vi "CFX.vi"(0 "CFX cmd":T6, 1 "CFX State":T7, 5 "CFX-config":T2={"neme"="上板机", "CFX Handle"="Cleaner", "Request IP"="amqp://192.168.1.10:5672", "User"="admin", "password"="123456", "Broker IP"="192.168.1.20", "Broker Port"="5672", "Publish Path"="/exchange/Cleaner", "SubPubish Path"="/queue/Broadcast-Cleaner", "Broadcast \nPublish Path"="/exchange/CFX.Host", "Broadcast Sub\npublish Path"="/queue/Broadcast-CFX.Host", "Target \nHandle lD"="CFX.Host", "target IP"="amqp://127.0.0.1", "unit verification"=TRUE, "heartbeat"=FALSE, "timeout period"=40.0}, 7 "CfxData":T1={"Vendor"="YXD", "UniqueIdentifier"="UID5620001", "FriendlyName"="SBJ", "ModelNumber"="SBJ_0001", "SerialNumber"="563210", "NumberofLanes"="2", "CodeIn"="", "CodeOut"="", "Unitldentifer"="", "PositionNumber"="", "PositionName"="", "OldState"="", "NewState"="", "OldStateDuration"="", "Faultcode"="", "Operatorldentifer"="", "LoginName"="", "RecipeName"="", "Revision"="", "Activate formula"="", "Description"=""}, 11 "Error In":errorcluster caption="错误输入", 12 "send?":bool) -> (6 "MessageCFX_out":string, 8 "CFX_Message_In":T3, 14 "ok?":bool, 15 "Error Out":errorcluster caption="错误输出")   [LabVIEW 2025]
uses:
  CFX_dll/CFX.dll
  ctl/CFX-cmd.ctl
  ctl/CfxTopic-cmd.ctl
  SubVI/table/1 model/a log/_myType runlog cmd.ctl
  ctl/CFX-config.ctl
  ctl/CFX_data.ctl
panel:
  out "QueueName":string
  out "IsOpenRequest":bool
  out "IsOpen":bool
  in  "CFX.Host?":bool
  in  "enable?":bool
  out "TraceMessage_EVE":refnum<k27>
  out "TraceMessage":string
  out "AooLog":refnum<k24>
  out "TestSubscribeChannel":bool
  out "TestPublishChannel":bool
  out "log":string
  out "error out":errorcluster
  out "objAMQP_MSG":refnum<k27>
  out "Connection":T4 {"ConnectionEstablished" items=["ConnectionEstablished", "ConnectionFailed", "ConnectionInterrupted", "ConnectionClosed"]}
  out "objAMQP_Request":refnum<k27>
  out "SubscribeChannel":refnum<k24>
  out "return":T5={"CFXHandle"="Cleaner", "RequestNetworkUri"="amqp://10.33.191.97:5672", "RequestTargetAddress"="/queue/Cleaner", "CFX_Message_In"={"Message_Name"="", "Message_Content"=""}, "CFX_Message_out"={"Message_Name"="", "Message_Content"=""}, "CFX_data"=refnum}
  out "FromListener":string
  in  "EndpointInformation":string
  in  "NewState":i32(ring)=1000 items=["PRD"=1000, "PRD_RegularWork"=1100, "PRD_WorkForThirdParties"=1200, "PRD_Rework"=1300, "PRD_Engineering"=1400, "SBY"=2000, "SBY_NoOperator"=2100, "SBY_NoProduct"=2200, "SBY_NoSupportTool"=2300, "SBY_AssociatedClusterModuleDown"=2400, "SBY_NoHost"=2500, "ENG"=3000, "ENG_ProcessExperiments"=3100, "ENG_EquipmentExperiments"=3200, "SDT"=4000, "SDT_UserMaintenanceDelay"=4100, "SDT_SuppliedMaintenanceDelay"=4200, "SDT_PreventiveMaintenance"=4300, "SDT_ChangeOfConsumables"=4400, "SDT_Setup"=4500, "SDT_ProductionTest"=4600, "SDT_FacilitiesRelated"=4700, "USD"=5000, "USD_UserMaintentanceDelay"=5100, "USD_SuppliedMaintenanceDelay"=5200, "USD_Repair"=5300, "USD_OutOfSpecInputMaterial"=5400, "USD_ChangeOfConsumables"=5500, "USD_FacilitiesRelated"=5600, "NST"=6000, "NST_UnworkedShifts"=6100, "NST_EquipmentInstallation"=6200, "NST_EquipmentModifications"=6300, "NST_OfflineTraining"=6400, "NST_ShutdownAndStartup"=6500]
  in  "Broker Url":string="amqp://admin:123456@10.33.191.54:5672"
  out "PublishChannel":refnum<k24>
  in  "rngNewState":i32(ring) items=["PRD"=1000, "PRD_RegularWork"=1100, "PRD_WorkForThirdParties"=1200, "PRD_Rework"=1300, "PRD_Engineering"=1400, "SBY"=2000, "SBY_NoOperator"=2100, "SBY_NoProduct"=2200, "SBY_NoSupportTool"=2300, "SBY_AssociatedClusterModuleDown"=2400, "SBY_NoHost"=2500, "ENG"=3000, "ENG_ProcessExperiments"=3100, "ENG_EquipmentExperiments"=3200, "SDT"=4000, "SDT_UserMaintenanceDelay"=4100, "SDT_SuppliedMaintenanceDelay"=4200, "SDT_PreventiveMaintenance"=4300, "SDT_ChangeOfConsumables"=4400, "SDT_Setup"=4500, "SDT_ProductionTest"=4600, "SDT_FacilitiesRelated"=4700, "USD"=5000, "USD_UserMaintentanceDelay"=5100, "USD_SuppliedMaintenanceDelay"=5200, "USD_Repair"=5300, "USD_OutOfSpecInputMaterial"=5400, "USD_ChangeOfConsumables"=5500, "USD_FacilitiesRelated"=5600, "NST"=6000, "NST_UnworkedShifts"=6100, "NST_EquipmentInstallation"=6200, "NST_EquipmentModifications"=6300, "NST_OfflineTraining"=6400, "NST_ShutdownAndStartup"=6500]
  # "此端点的唯一 CFX 句柄。"
  # "节点队列名"
  # "amqp://10.33.191.64:5672"
  # "amqp://localhost:5672"
  # "Laser"
  # "amqp://192.168.1.20:5672"
  # "AMQP 源或目标的网络地址。可以包括 user 和 port 信息 标准 Uri 格式。（例如：amqps://user1:password1@myamqpbroker.company1.com、amqp://broker3.company1.com、 amqps://myamqpbroker.company1.com:8856 等）。"
  # "本地消息源\nRequest Source"
  # "代理层\nBroker"
  # "请求目标\nRequest Target"
  # "可配置项"
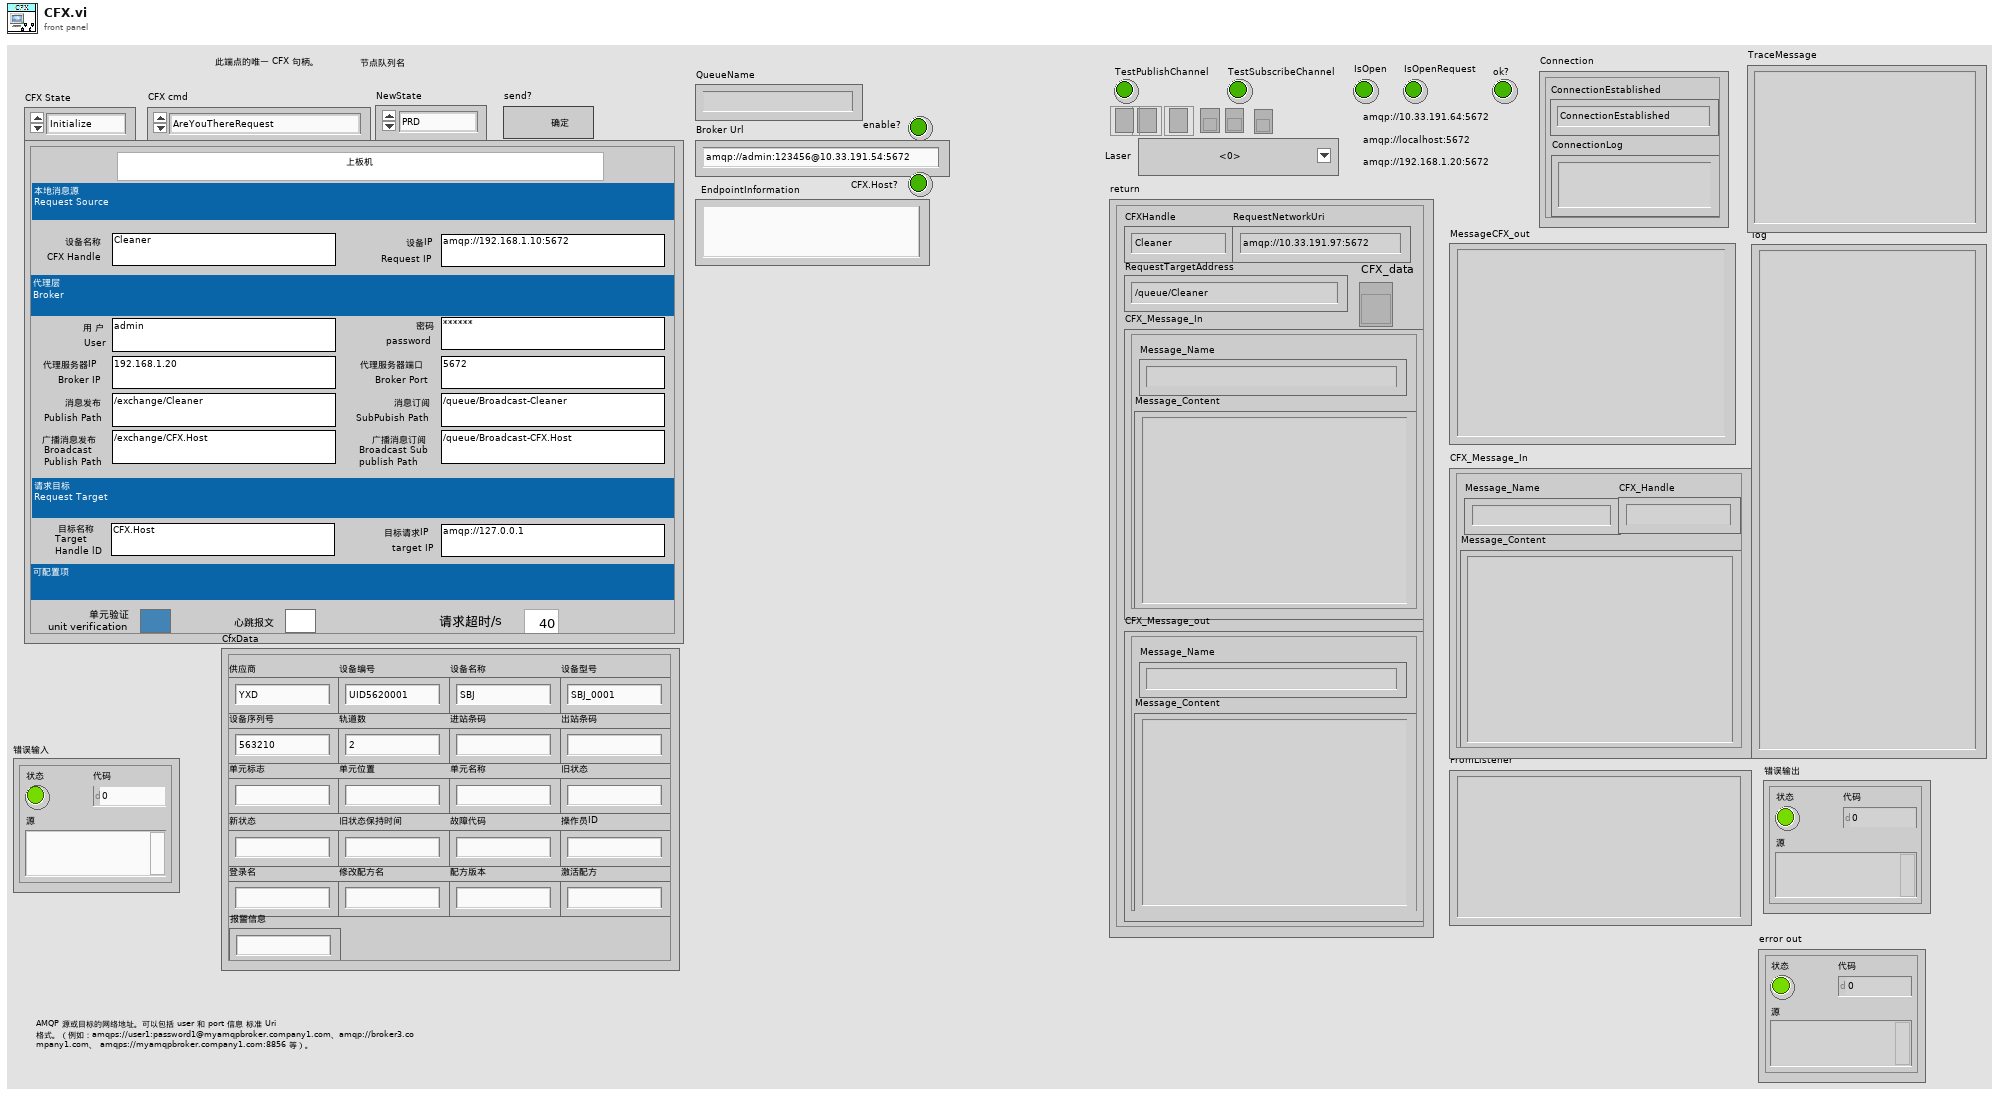
[diagram p1: front panel]
types:
  T1 = typedef "CFX_data.ctl" = cluster{"Vendor":string, "UniqueIdentifier":string, "FriendlyName":string, "ModelNumber":string, "SerialNumber":string, "NumberofLanes":string, "CodeIn":string, "CodeOut":string, "Unitldentifer":string, "PositionNumber":string, "PositionName":string, "OldState":string, "NewState":string, "OldStateDuration":string, "Faultcode":string, "Operatorldentifer":string, "LoginName":string, "RecipeName":string, "Revision":string, "Activate formula":string, "Description":string}
  T2 = typedef "CFX-config.ctl" = cluster{"neme":string, "CFX Handle":string, "Request IP":string, "User":string, "password":string, "Broker IP":string, "Broker Port":string, "Publish Path":string, "SubPubish Path":string, "Broadcast \nPublish Path":string, "Broadcast Sub\npublish Path":string, "Target \nHandle lD":string, "target IP":string, "unit verification":bool, "heartbeat":bool, "timeout period":dbl}
  T3 = cluster{"Message_Name":string, "CFX_Handle":string, "Message_Content":string}
  T4 = cluster{"ConnectionEstablished":i32, "ConnectionLog":string}
  T5 = cluster{"CFXHandle":string, "RequestNetworkUri":string, "RequestTargetAddress":string, "CFX_Message_In":cluster{"Message_Name":string, "Message_Content":string}, "CFX_Message_out":cluster{"Message_Name":string, "Message_Content":string}, "CFX_data":refnum<vi>}
  T6 = typedef "CfxTopic-cmd.ctl" = enum16{"AreYouThereRequest", "AreYouThereResponse", "EndpointConnected", "EndpointShuttingDown", "GetEndpointInformationRequest", "GetEndpointInformationResponse", "Heartbeat", "NotSupportedResponse", "WhoIsThereRequest", "WhoIsThereResponse", "UnitArrived", "UnitsDeparted", "StationStateChanged", "FaultOccurred", "FaultCleared", "OperatorActivated", "OperatorDeactivated", "RecipeModified", "RecipeActived", "ActivateRecipeRequest", "ActivateRecipeResponse"}
  T7 = typedef "CFX-cmd.ctl" = enum16{"Initialize", "Event", "Connection test", "OpenConnection", "Idle", "Shutdown", "WorkComplete", "StationStateChanged", "MaterialsApplied", "CFX", "Hermes"}
  T8 = typedef "_myType runlog cmd.ctl" = enum16{"init", "push (-1: error)", "push (0: user)", "push (1: logical)", "push (2: driver)", "push (3: lib-core)", "push (4: reserved)", "pop", "more?"}
  T9 = typedef "LVStringsAndValuesArrayTypeDef_I32.ctl" = cluster{"String":string, "Value":i32}[]
  T10 = cluster{"Message_Name":string, "Message_Content":string}
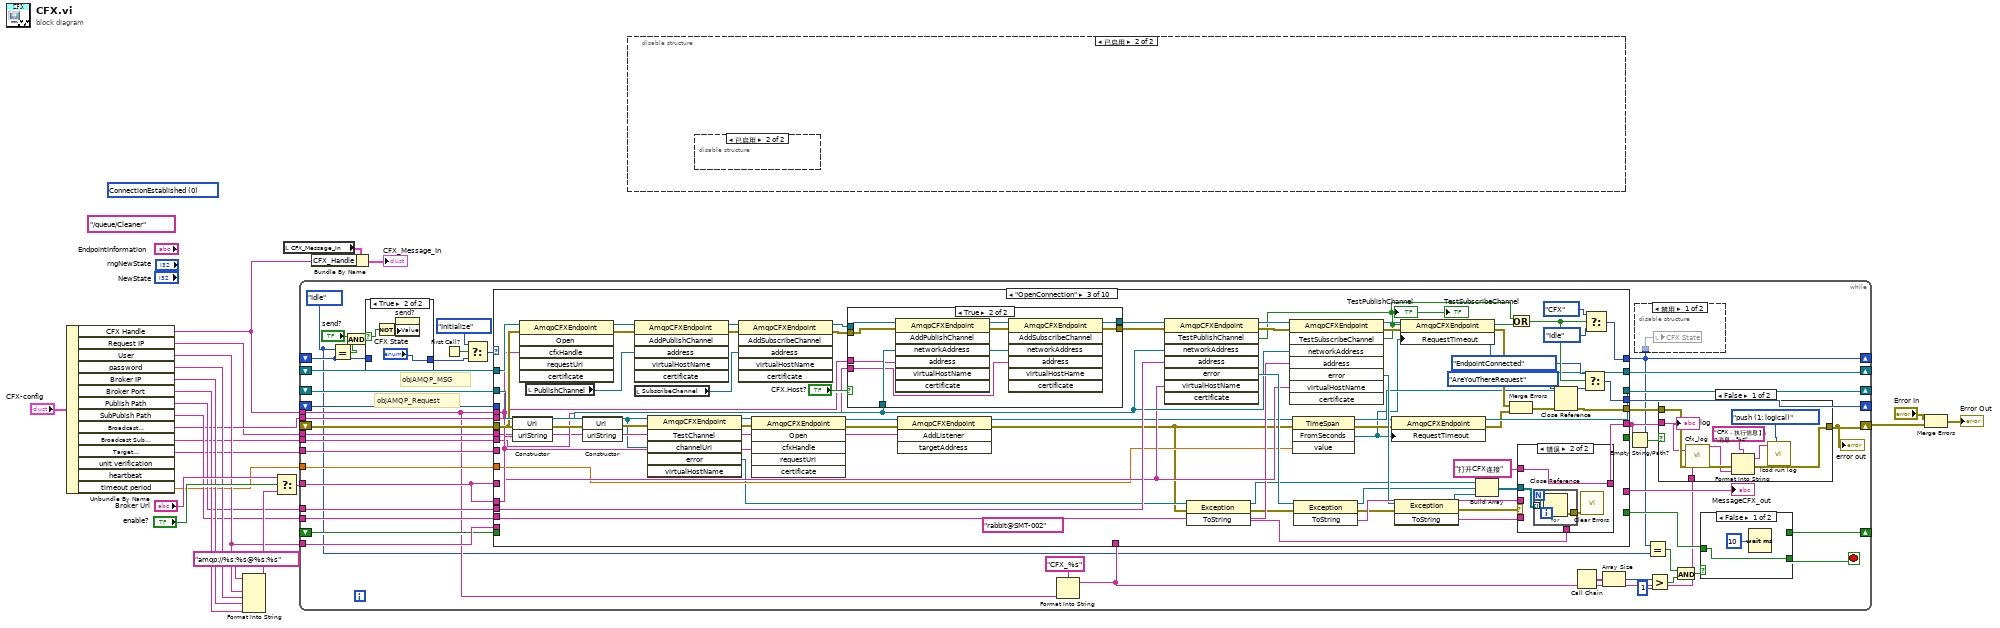
[diagram p0: block diagram]
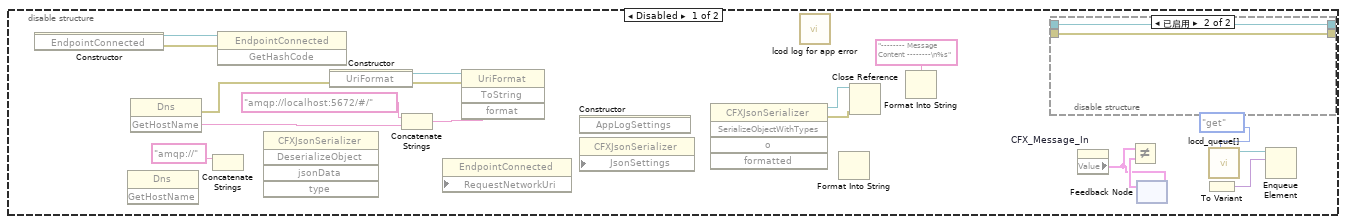
[diagram p2: hidden frame]
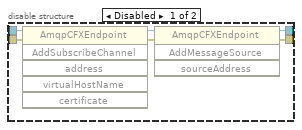
[diagram p3: hidden frame]
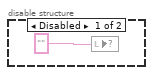
[diagram p4: hidden frame]
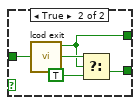
[diagram p7: hidden frame]
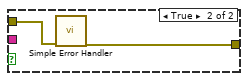
[diagram p8: hidden frame]
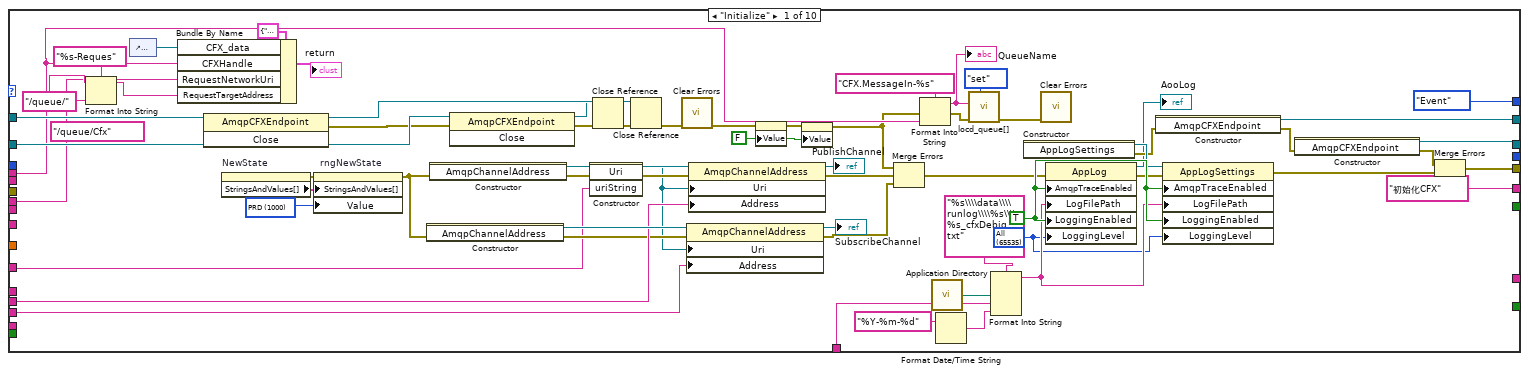
[diagram p9: hidden frame]
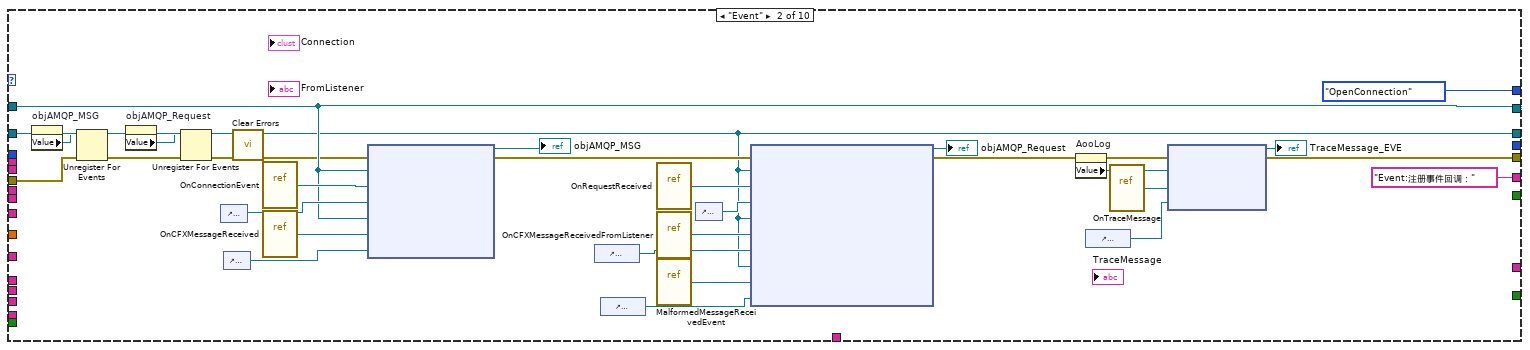
[diagram p10: hidden frame]
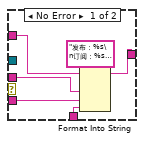
[diagram p12: hidden frame]
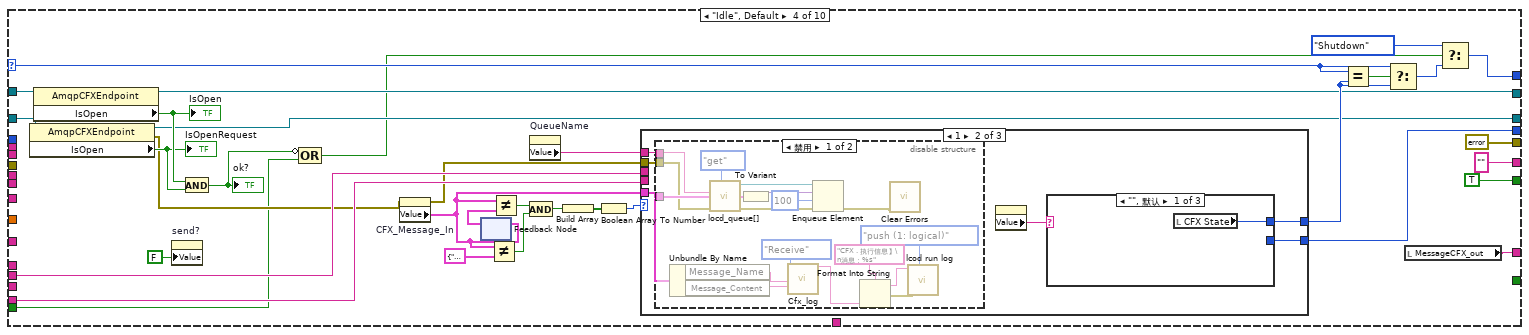
[diagram p13: hidden frame]
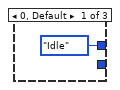
[diagram p14: hidden frame]
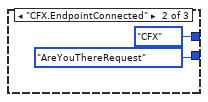
[diagram p16: hidden frame]
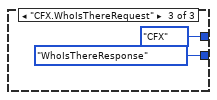
[diagram p17: hidden frame]
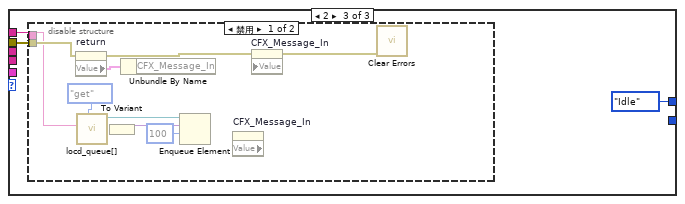
[diagram p18: hidden frame]
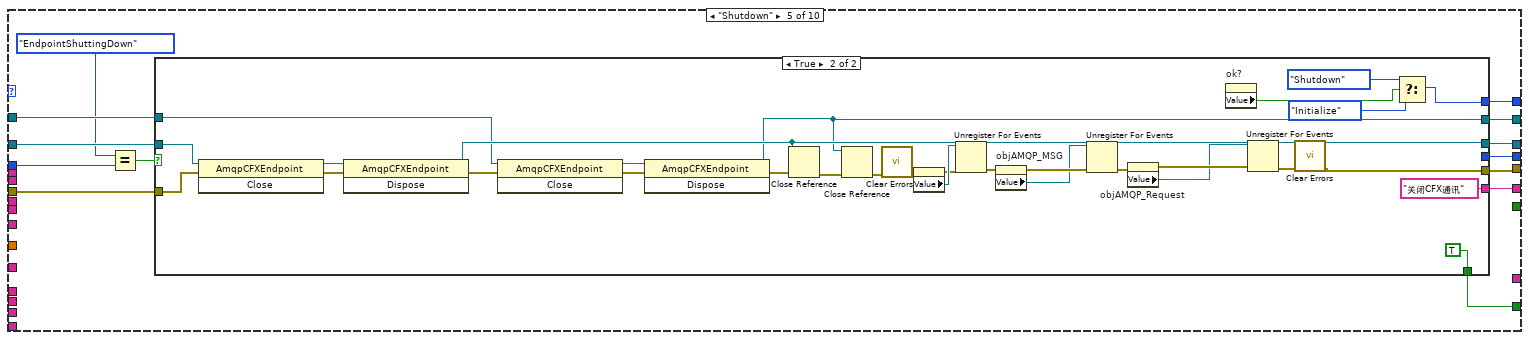
[diagram p20: hidden frame]
diagram:
  (unwired) "/queue/Cleaner" ("RequestTargetAddress")
  (unwired) 0 items=["ConnectionEstablished", "ConnectionFailed", "ConnectionInterrupted", "ConnectionClosed"] ("ConnectionEstablished")
  n1 = Unbundle By Name("CFX-config") -> ("CFX Handle"=w3:string, "Request IP"=w6:string, "User"=w16:string, "password"=w15:string, "Broker IP"=w14:string, "Broker Port"=w13:string, "Publish Path"=w12:string, "SubPubish Path"=w11:string, "Broadcast \nPublish Path"=w10:string, "Broadcast Sub\npublish Path"=w9:string, "Target \nHandle lD"=w8:string, "timeout period"=w7:dbl)  [unwired: 2 out]
  n2 = Format Into String(format string="amqp://%s:%s@%s:%s" ("格式字符串"), w16, w15, w14, w13) -> (resulting string=w18:string)  [unwired: 2 in, 1 out]
  n3 = Select(t="Broker Url", s="enable?", f=w18) -> (s? t:f=w5:string)
  n4 = local read "CFX_Message_In"() -> (w2:T3)
  n5 = while {
    shift-right: [w41] -> _
    shift-left: _ -> [w27]
    shift-right: [w66] -> _
    shift-left: _ -> [w67]
    shift-right: [w63] -> _
    shift-left: _ -> [w62]
    shift-right: [w58] -> w4
    shift-left: _ -> [w52]
    shift-right: [w57] -> _
    shift-left: _ -> [w59]
    tunnel: w5 -> [w53]
    tunnel: w11 -> [w56]
    tunnel: w12 -> [w55]
    tunnel: w3 -> [w32]
    tunnel: w16 -> [w54]
    tunnel: w6 -> [w51]
    tunnel: w10 -> [w50]
    tunnel: w9 -> [w49]
    tunnel: w8 -> [w48]
    tunnel: w7 -> [w47]
    shift-right: [w28] -> _
    shift-left: _ -> [w34]
    stop <- w42 stop-if-true
    w26 = CFX-cmd."Idle" ("CFX State")
    # "objAMQP_Request"
    # "objAMQP_MSG"
    n6 = Equal?(x=w26, y=w27) -> (x = y?=w24:bool)
    n7 = And(x="send?", y=w24) -> (x .and. y?=w25:bool)
    n8 = case shown="True" w25 {
      selector: w25 -> [_ w71]
      tunnel: w27 -> [w69 _]
      tunnel: [w69 "CFX State"] -> w31
      frame False {
      }
      frame True {
        n9 = Not(x=w71) -> (.not. x?=w70:bool)
        n10 = property on="send?" class="Bool (严格)"("Value"=w70) -> ()  [unwired: 2 in, 2 out]
      }
    }
    n11 = First Call?() -> (First Call?: T/F=w36:bool)
    n12 = Select(t=CFX-cmd."Initialize" ("CFX State"), s=w36, f=w31) -> (s? t:f=w35:T7)
    n13 = Format Into String(format string="CFX_%s" ("log_path"), w32) -> (resulting string=w30:string)  [unwired: 2 in, 1 out]
    n14 = case shown="\"OpenConnection\"" w35 {
      selector: w35 -> [_ _ _ w306 _ _ _ _ _ _]
      tunnel: [_ _ _ _ w352 _ _ _ _ _] -> w43
      tunnel: w67 -> [w131 w161 w250 w294 w360 w412 w441 w467 w508 w527]
      tunnel: [w138 w161 w203 w293 w355 w411 w439 w466 w506 w526] -> w66
      tunnel: [w132 w173 w217 errorcluster {"status"=FALSE, "code"=0, "source"=""} ("error out") w353 w408 w436 w465 w518 w525] -> w65
      tunnel: [_ _ _ w305 _ w403 w428 w452 w501 w524] -> w64
      tunnel: [_ _ _ TRUE _ _ _ _ _ _] -> _
      tunnel: ["初始化CFX" ("格式字符串") "Event:注册事件回调：" ("SerializeObjectWithTypes") w242 "" ("SerializeObjectWithTypes") w359 w400 w428 w451 w512 w524] -> w61
      tunnel: [CFX-cmd."Event" ("CFX State") CFX-cmd."OpenConnection" ("CFX State") w210 w284 w358 CFX-cmd."Idle" ("CFX State") CFX-cmd."Idle" ("CFX State") CFX-cmd."Idle" ("CFX State") w487 CFX-cmd."Idle" ("CFX State")] -> w41
      tunnel: [w137 w160 w234 w288 w354 w397 w425 w448 w507 w521] -> w63
      tunnel: w62 -> [w130 w160 w246 w295 w356 w397 w425 w448 w507 w521]
      tunnel: w52 -> [_ w168 w221 _ w357 w398 w426 w449 w509 w522]
      tunnel: w59 -> [_ _ _ _ w351 _ _ _ w491 _]
      tunnel: [_ _ w206 w300 w348 _ _ _ w486 _] -> w57
      tunnel: w53 -> [w93 _ _ _ _ _ _ _ _ _]
      tunnel: w56 -> [w117 _ w199 _ _ _ _ _ _ _]
      tunnel: w55 -> [w116 _ w230 w297 _ _ _ _ _ _]
      tunnel: w32 -> [w96 _ w213 _ _ _ _ _ w484 _]
      tunnel: w54 -> [_ _ _ w296 _ _ _ _ _ _]
      tunnel: w53 -> [_ _ w229 _ _ _ _ _ _ _]
      tunnel: w51 -> [w97 _ w196 _ _ _ _ _ _ _]
      tunnel: w50 -> [_ _ w201 _ _ _ _ _ _ _]
      tunnel: w49 -> [_ _ w200 _ _ _ _ _ _ _]
      tunnel: w48 -> [_ _ _ _ _ _ _ _ w483 _]
      tunnel: w47 -> [_ _ w198 _ _ _ _ _ _ _]
      tunnel: w34 -> [_ _ _ w287 _ _ _ _ _ _]
      tunnel: w30 -> [w95 _ _ _ _ _ _ _ _ _]
      frame "Initialize" {
        (unwired) "/queue/Cfx" ("RequestTargetAddress")
        w121 = FALSE ("TestPublishChannel")
        w134 = 65535 items=["Debug"=1, "Info"=2, "Warn"=4, "Error"=8, "All"=65535] ("LoggingLevel")
        w136 = TRUE ("LoggingEnabled")
        w149 = 1000 items=["PRD"=1000, "PRD_RegularWork"=1100, "PRD_WorkForThirdParties"=1200, "PRD_Rework"=1300, "PRD_Engineering"=1400, "SBY"=2000, "SBY_NoOperator"=2100, "SBY_NoProduct"=2200, "SBY_NoSupportTool"=2300, "SBY_AssociatedClusterModuleDown"=2400, "SBY_NoHost"=2500, "ENG"=3000, "ENG_ProcessExperiments"=3100, "ENG_EquipmentExperiments"=3200, "SDT"=4000, "SDT_UserMaintenanceDelay"=4100, "SDT_SuppliedMaintenanceDelay"=4200, "SDT_PreventiveMaintenance"=4300, "SDT_ChangeOfConsumables"=4400, "SDT_Setup"=4500, "SDT_ProductionTest"=4600, "SDT_FacilitiesRelated"=4700, "USD"=5000, "USD_UserMaintentanceDelay"=5100, "USD_SuppliedMaintenanceDelay"=5200, "USD_Repair"=5300, "USD_OutOfSpecInputMaterial"=5400, "USD_ChangeOfConsumables"=5500, "USD_FacilitiesRelated"=5600, "NST"=6000, "NST_UnworkedShifts"=6100, "NST_EquipmentInstallation"=6200, "NST_EquipmentModifications"=6300, "NST_OfflineTraining"=6400, "NST_ShutdownAndStartup"=6500] ("NewState")
        n15 = Format Into String(format string="%s-Reques" ("格式字符串"), initial string="/queue/" ("RequestTargetAddress"), w96) -> (resulting string=w90:string)  [unwired: 1 in, 1 out]
        n16 = control-ref of="CfxData"() -> (w101:refnum<vi>)
        n17 = Bundle By Name(cluster=T5 {"CFXHandle"="Cleaner", "RequestNetworkUri"="amqp://192.168.1.10:5672", "RequestTargetAddress"="/queue/Cleaner", "CFX_Message_In"={"Message_Name"="", "Message_Content"=""}, "CFX_Message_out"={"Message_Name"="", "Message_Content"=""}, "CFX_data"=refnum} ("return"), "CFX_data"=w101, "CFXHandle"=w96, "RequestNetworkUri"=w97, "RequestTargetAddress"=w90) -> (→"return":T5)
        n18 = invoke class="AmqpCFXEndpoint" method="Close"(reference=w131) -> (reference out=w125:refnum<k24>, error out=w129:errorcluster)  [unwired: 2 in, 1 out]
        n19 = property on="NewState" class="Ring (严格)"() -> (error out=w148:errorcluster, "StringsAndValues[]"=w152:T9)  [unwired: 2 in, 1 out]
        n20 = property on="rngNewState" class="Ring (严格)"(error in=w148, "StringsAndValues[]"=w152, "Value"=w149) -> (error out=w123:errorcluster)  [unwired: 1 in, 1 out]
        n21 = constructor class="AmqpChannelAddress"(error in=w123) -> (reference out=w142:refnum<k24>, error out=w115:errorcluster)  [unwired: 2 in, 1 out]
        n22 = constructor class="AmqpChannelAddress"(error in=w123) -> (reference out=w147:refnum<k24>, error out=w151:errorcluster)  [unwired: 2 in, 1 out]
        n23 = invoke class="AmqpCFXEndpoint" method="Close"(reference=w130, error in=w129) -> (reference out=w124:refnum<k24>, error out=w128:errorcluster)  [unwired: 1 in, 1 out]
        n24 = constructor class="Uri"(error in=w151, "uriString"=w93) -> (reference out=w114:refnum<k24>, error out=w150:errorcluster)  [unwired: 2 in, 2 out]
        n25 = Close Reference(reference=w124, error in (no error)=w128) -> (error out=w127:errorcluster)
        n26 = Close Reference(reference=w125, error in (no error)=w127) -> (error out=w126:errorcluster)
        n27 = call <vilib>:"Clear Errors.vi"("error in (no error)"=w126) -> ("error out"=w113:errorcluster)  [unwired: 5 in, 1 out]
        n28 = property class="AmqpChannelAddress"(reference=w142, error in=w115, "Uri"=w114, "Address"=w117) -> (reference out=→"SubscribeChannel":refnum<k24>, error out=w140:errorcluster)
        n29 = property class="AmqpChannelAddress"(reference=w147, error in=w150, "Uri"=w114, "Address"=w116) -> (reference out=→"PublishChannel":refnum<k24>, error out=w141:errorcluster)
        n30 = property on="TestPublishChannel" class="Bool (严格)"(error in=w113, "Value"=w121) -> (error out=w122:errorcluster)  [unwired: 1 in, 1 out]
        n31 = property on="TestSubscribeChannel" class="Bool (严格)"(error in=w122, "Value"=w121) -> (error out=w92:errorcluster)  [unwired: 1 in, 1 out]
        n32 = Merge Errors(w92, w141, w140) -> (w104:errorcluster)
        n33 = Format Into String(format string="CFX.MessageIn-%s" ("格式字符串"), error in=w92, w96) -> (resulting string=w105:string, error out=w102:errorcluster)  [unwired: 1 in]
        "QueueName" <- w105
        n34 = call <vilib>:"Application Directory.vi"() -> ("Application Directory"=w146:path)
        n35 = Format Date/Time String(time format string (%c)="%Y-%m-%d" ("格式字符串")) -> (date/time string=w94:string)  [unwired: 2 in]
        n36 = call "locd_queue[].vi"("cmd"=enum16{"init", "get", "set", "end"}."set", "error in"=w102, "queue_name"=w105) -> ("error out"=w103:errorcluster)  [unwired: 4 in, 4 out]
        n37 = Format Into String(format string="%s\\\\data\\\\runlog\\\\%s\\\\%s_cfxDebig.txt" ("格式字符串"), w146, w95, w94) -> (resulting string=w135:string)  [unwired: 2 in, 1 out]
        n38 = constructor class="AppLogSettings"() -> (reference out=w133:refnum<k24>, error out=w120:errorcluster)  [unwired: 3 in, 1 out]
        n39 = call <vilib>:"Clear Errors.vi"("error in (no error)"=w103) -> ()  [unwired: 5 in, 2 out]
        n40 = property class="AppLog"(error in=w104, "AmqpTraceEnabled"=w136, "LogFilePath"=w135, "LoggingEnabled"=w136, "LoggingLevel"=w134) -> (reference out=→"AooLog":refnum<k24>, error out=w118:errorcluster)  [unwired: 1 in]
        n41 = constructor class="AmqpCFXEndpoint"(error in=w120) -> (reference out=w138:refnum<k24>, error out=w109:errorcluster)  [unwired: 2 in, 1 out]
        n42 = property class="AppLogSettings"(reference=w133, error in=w118, "AmqpTraceEnabled"=w136, "LogFilePath"=w135, "LoggingEnabled"=w136, "LoggingLevel"=w134) -> (error out=w110:errorcluster)  [unwired: 1 out]
        n43 = constructor class="AmqpCFXEndpoint"(error in=w109) -> (reference out=w137:refnum<k24>, error out=w108:errorcluster)  [unwired: 2 in, 1 out]
        n44 = Merge Errors(w108, w110) -> (w132:errorcluster)
      }
      frame "Event" {
        n45 = property on="objAMQP_MSG" class="Ref (严格)"() -> ("Value"=w155:refnum<k27>)  [unwired: 2 in, 2 out]
        n46 = Unregister For Events(event registration refnum=w155, error in=w168) -> (error out=w156:errorcluster)
        n47 = property on="objAMQP_Request" class="Ref (严格)"() -> ("Value"=w153:refnum<k27>)  [unwired: 2 in, 2 out]
        n48 = Unregister For Events(event registration refnum=w153, error in=w156) -> (error out=w154:errorcluster)
        n49 = control-ref of="Connection"() -> (w180:refnum<vi>)
        n50 = control-ref of="CFX_Message_In"() -> (w165:refnum<vi>)
        n51 = call <vilib>:"Clear Errors.vi"("error in (no error)"=w154) -> ("error out"=w157:errorcluster)  [unwired: 5 in, 1 out]
        n52 = vi-ref "OnConnectionEvent.vi"() -> ("vi reference"=w181:refnum<vi>)
        n53 = vi-ref "OnCFXMessageReceived.vi"() -> ("vi reference"=w166:refnum<vi>)
        n54 = node(w157, w161, w181, w180, w161, w166, w165) -> (→"objAMQP_MSG":refnum<k27>, w164:errorcluster)  [unwired: 1 in]
        n55 = control-ref of="FromListener"() -> (w162:refnum<vi>)
        n56 = control-ref of="FromListener"() -> (w158:refnum<vi>)
        n57 = vi-ref "OnRequestReceived.vi"() -> ("vi reference"=w179:refnum<vi>)
        n58 = vi-ref "OnCFXMessageReceivedFromListener.vi"() -> ("vi reference"=w163:refnum<vi>)
        n59 = vi-ref "MalformedMessageReceivedEvent.vi"() -> ("vi reference"=w159:refnum<vi>)
        n60 = control-ref of="return"() -> (w170:refnum<vi>)
        n61 = node(w164, w160, w179, w170, w160, w163, w162, w160, w159, w158) -> (→"objAMQP_Request":refnum<k27>, w167:errorcluster)  [unwired: 1 in]
        n62 = property on="AooLog" class="Ref (严格)"(error in=w167) -> (error out=w169:errorcluster, "Value"=w175:refnum<k24>)  [unwired: 1 in, 1 out]
        n63 = control-ref of="TraceMessage"() -> (w171:refnum<vi>)
        n64 = vi-ref "OnTraceMessage.vi"() -> ("vi reference"=w174:refnum<vi>)
        n65 = node(w169, w175, w174, w171) -> (→"TraceMessage_EVE":refnum<k27>, w173:errorcluster)  [unwired: 1 in]
      }
      frame "OpenConnection" {
        (unwired) "rabbit@SMT-002" ("sourceAddress")
        n66 = constructor class="Uri"(error in=w221, "uriString"=w229) -> (reference out=w228:refnum<k24>, error out=w226:errorcluster)  [unwired: 2 in, 2 out]
        n67 = invoke class="AmqpCFXEndpoint" method="Open"(reference=w250, error in=w221, "cfxHandle"=w213) -> (reference out=w225:refnum<k24>, error out=w224:errorcluster)  [unwired: 3 in, 4 out]
        n68 = local read "PublishChannel"() -> (w244:refnum<k24>)
        n69 = constructor class="Uri"(error in=w226, "uriString"=w196) -> (reference out=w183:refnum<k24>, error out=w194:errorcluster)  [unwired: 2 in, 2 out]
        n70 = local read "SubscribeChannel"() -> (w245:refnum<k24>)
        n71 = invoke class="AmqpCFXEndpoint" method="AddPublishChannel"(reference=w225, error in=w224, "address"=w244) -> (reference out=w249:refnum<k24>, error out=w248:errorcluster)  [unwired: 3 in, 4 out]
        n72 = invoke on="调用节点" class="AmqpCFXEndpoint" method="TestChannel"(reference=w246, error in=w194, "channelUri"=w183) -> (reference out=w185:refnum<k24>, error out=w184:errorcluster, "error"=w193:refnum<k24>)  [unwired: 3 in, 3 out]
        n73 = invoke class="AmqpCFXEndpoint" method="AddSubscribeChannel"(reference=w249, error in=w248, "address"=w245) -> (reference out=w222:refnum<k24>, error out=w214:errorcluster)  [unwired: 3 in, 4 out]
        n74 = invoke class="AmqpCFXEndpoint" method="Open"(reference=w185, error in=w184, "cfxHandle"=w213, "requestUri"=w183) -> (reference out=w231:refnum<k24>, error out=w195:errorcluster)  [unwired: 2 in, 4 out]
        n75 = case shown="True" "CFX.Host?" {
          tunnel: w228 -> [_ w261]
          tunnel: [w251 w260] -> w227
          tunnel: [w252 w259] -> w223
          tunnel: w222 -> [w252 w258]
          tunnel: w214 -> [w251 w255]
          tunnel: w201 -> [_ w254]
          tunnel: w200 -> [_ w253]
          frame False {
          }
          frame True {
            n76 = invoke class="AmqpCFXEndpoint" method="AddPublishChannel"(reference=w258, error in=w255, "networkAddress"=w261, "address"=w254) -> (reference out=w256:refnum<k24>, error out=w257:errorcluster)  [unwired: 3 in, 5 out]
            n77 = invoke class="AmqpCFXEndpoint" method="AddSubscribeChannel"(reference=w256, error in=w257, "networkAddress"=w261, "address"=w253) -> (reference out=w259:refnum<k24>, error out=w260:errorcluster)  [unwired: 3 in, 5 out]
          }
        }
        n78 = invoke on="调用节点" class="AmqpCFXEndpoint" method="AddListener"(reference=w231, error in=w195, "targetAddress"=w196) -> (reference out=w197:refnum<k24>, error out=w192:errorcluster)  [unwired: 1 in, 2 out]
        n79 = invoke on="调用节点" class="AmqpCFXEndpoint" method="TestPublishChannel"(reference=w223, error in=w227, "networkAddress"=w228, "address"=w230, "virtualHostName"=w213) -> (reference out=w243:refnum<k24>, error out=w233:errorcluster, "TestPublishChannel"=w212:bool, "error"=w240:refnum<k24>)  [unwired: 3 in, 4 out]
        "TestPublishChannel" <- w212
        n80 = invoke class="Exception" method="ToString"(reference=w193, error in=w192) -> (reference out=w189:refnum<k24>, error out=w191:errorcluster, "ToString"=w190:string)  [unwired: 1 in]
        n81 = invoke on="调用节点" class="AmqpCFXEndpoint" method="TestSubscribeChannel"(reference=w243, error in=w233, "networkAddress"=w228, "address"=w199, "virtualHostName"=w213) -> (reference out=w241:refnum<k24>, error out=w219:errorcluster, "TestSubscribeChannel"=w211:bool, "error"=w237:refnum<k24>)  [unwired: 3 in, 4 out]
        "TestSubscribeChannel" <- w211
        n82 = invoke class="TimeSpan" method="FromSeconds"(error in=w192, "value"=w198) -> (reference out=w216:refnum<k24>, error out=w218:errorcluster, "FromSeconds"=w202:refnum<k24>)  [unwired: 2 in, 1 out]
        n83 = invoke class="Exception" method="ToString"(reference=w240, error in=w191) -> (reference out=w188:refnum<k24>, error out=w238:errorcluster, "ToString"=w239:string)  [unwired: 1 in]
        n84 = property on="属性节点" class="AmqpCFXEndpoint"(reference=w197, error in=w218, "RequestTimeout"=w202) -> (reference out=w234:refnum<k24>, error out=w220:errorcluster)
        n85 = invoke class="Exception" method="ToString"(reference=w237, error in=w238) -> (reference out=w187:refnum<k24>, error out=w235:errorcluster, "ToString"=w236:string)  [unwired: 1 in]
        n86 = property on="属性节点" class="AmqpCFXEndpoint"(reference=w241, "RequestTimeout"=w202) -> (reference out=w203:refnum<k24>)  [unwired: 1 in, 1 out]
        n87 = Build Array(w189, w188, w187) -> (w186:refnum<k24>[])
        n88 = Merge Errors(w219, w220) -> (w232:errorcluster)
        n89 = Or(x=w212, y=w211) -> (x .or. y?=w207:bool)
        n90 = case shown="错误" w235 {
          tunnel: "打开CFX连接" ("格式字符串") -> [w267 w270]
          tunnel: [w266 w270] -> w242
          tunnel: w239 -> [w264 _]
          tunnel: w236 -> [w263 _]
          tunnel: w190 -> [w262 _]
          tunnel: w186 -> [_ w269]
          frame No Error {
            n91 = Format Into String(format string="发布：%s\n订阅：%s\n监听监控：%s" ("格式字符串"), initial string=w267, w264, w263, w262) -> (resulting string=w266:string)  [unwired: 1 in, 1 out]
          }
          frame Error {
            n92 = for {
              tunnel: w269 -> [w272] mode=indexing
              tunnel: [w271] -> w268
              n93 = Close Reference(reference=w272) -> (error out=w271:errorcluster)  [unwired: 1 in]
            }
            n94 = call <vilib>:"Clear Errors.vi"("error in (no error)"=w268) -> ()  [unwired: 5 in, 2 out]
          }
        }
        n95 = Close Reference(reference=w216, error in (no error)=w232) -> (error out=w217:errorcluster)
        n96 = Select(t=CfxTopic-cmd."EndpointConnected" ("CFX cmd"), s=w207, f=CfxTopic-cmd."AreYouThereRequest") -> (s? t:f=w206:T6)
        n97 = Select(t=CFX-cmd."CFX" ("CFX State"), s=w207, f=CFX-cmd."Idle" ("CFX State")) -> (s? t:f=w210:T7)
      }
      frame "Idle", Default {
        n98 = property on="属性节点" class="AmqpCFXEndpoint"(reference=w295) -> (reference out=w288:refnum<k24>, error out=w290:errorcluster, "IsOpen"=w291:bool)  [unwired: 1 in]
        "IsOpenRequest" <- w291
        n99 = property on="属性节点" class="AmqpCFXEndpoint"(reference=w294) -> (reference out=w293:refnum<k24>, "IsOpen"=w292:bool)  [unwired: 1 in, 1 out]
        "IsOpen" <- w292
        n100 = property on="send?" class="Bool (严格)"("Value"=FALSE ("send?")) -> ()  [unwired: 2 in, 2 out]
        n101 = And(x=w292, y=w291) -> (x .and. y?=w273:bool)
        "ok?" <- w273
        n102 = Compound Arithmetic op=OR ("复合运算")(invert w273, w287) -> (w274:bool)
        n103 = property on="CFX_Message_In" class="Clust (严格)"(error in=w290) -> (error out=w289:errorcluster, "Value"=w279:T3)  [unwired: 1 in, 1 out]
        n104 = feedback-in #1(w279) -> ()
        n105 = feedback #1() -> (w298:T3)  [unwired: 1 in]
        n106 = Not Equal?(x=w279, y=T3 {"Message_Name"="", "CFX_Handle"="", "Message_Content"=""} ("CFX_Message_In")) -> (x != y?=w277:bool)
        n107 = Not Equal?(x=w279, y=w298) -> (x != y?=w283:bool)
        n108 = And(x=w283, y=w277) -> (x .and. y?=w278:bool)
        n109 = property on="QueueName" class="Str"() -> ("Value"=w280:string)  [unwired: 2 in, 2 out]
        n110 = Build Array(w278) -> (w281:bool[])
        n111 = Boolean Array To Number(Boolean array=w281) -> (number=w282:u32)
        n112 = case shown="1" w282 {
          tunnel: [_ w313 _] -> w300
          tunnel: [CFX-cmd."Idle" ("CFX State") w312 CFX-cmd."Idle" ("CFX State")] -> w299
          tunnel: w297 -> [_ _ _]
          tunnel: w296 -> [_ _ _]
          tunnel: w279 -> [_ w310 _]
          tunnel: w289 -> [_ w308 w338]
          tunnel: w280 -> [_ w309 w336]
          frame 0, Default {
          }
          frame 1 {
            n113 = disable-structure shown="禁用" {
              disable-tunnel: w310 -> [w326 _]
              disable-tunnel: w309 -> [w316 _]
              disable-tunnel: w308 -> [w315 _]
              frame Disabled {
                n114 = Unbundle By Name(w326) -> ("Message_Name"=w325:string, "Message_Content"=w324:string)
                n115 = call "locd_queue[].vi"("cmd"=enum16{"init", "get", "set", "end"}."get", "error in"=w315, "queue_name"=w316) -> ("error out"=w327:errorcluster, "queue_out"=w329:refnum<queue>)  [unwired: 4 in, 3 out]
                n116 = To Variant(anything=w326) -> (Variant=w328:variant)
                n117 = call "Cfx_log.vi"("R/W"=enum16{"Send", "Receive"}."Receive", "Message_Name"=w325, "Message_Content"=w324) -> ("Log_out"=w318:string)  [unwired: 15 in, 1 out]
                n118 = Enqueue Element(queue=w329, element=w328, timeout in ms (-1)=100 ("超时毫秒(-1)"), error in (no error)=w327) -> (error out=w314:errorcluster)  [unwired: 2 out]
                n119 = Format Into String(format string="CFX . 执行信息】\n消息：%s", w318) -> (resulting string=w321:string, error out=w322:errorcluster)  [unwired: 2 in]
                n120 = call <vilib>:"Clear Errors.vi"("error in (no error)"=w314) -> ()  [unwired: 5 in, 2 out]
                n121 = call "lcod run log.vi"("cmd"=_myType_runlog_cmd."push (1: logical)", "Error In"=w322, "str in"=w321) -> ()  [unwired: 6 in, 3 out]
              }
              frame Enabled {
              }
            }
            n122 = property on="Message_Name" class="Str"() -> ("Value"=w311:string)  [unwired: 2 in, 2 out]
            n123 = case shown="\"\", 默认" w311 {
              tunnel: [_ CfxTopic-cmd."AreYouThereRequest" ("CFX cmd") CfxTopic-cmd."WhoIsThereResponse" ("CFX cmd")] -> w313
              tunnel: [w331 CFX-cmd."CFX" ("CFX State") CFX-cmd."CFX" ("CFX State")] -> w312
              frame "", Default {
                n124 = local read "CFX State"() -> (w331:T7)
              }
              frame "CFX.EndpointConnected" {
              }
              frame "CFX.WhoIsThereRequest" {
              }
            }
          }
          frame 2 {
            n125 = disable-structure shown="禁用" {
              disable-tunnel: w338 -> [w344 _]
              disable-tunnel: w336 -> [w339 _]
              frame Disabled {
                n126 = property on="return" class="Clust (严格)"(error in=w344) -> (error out=w346:errorcluster, "Value"=w345:T5)  [unwired: 1 in, 1 out]
                n127 = call "locd_queue[].vi"("cmd"=enum16{"init", "get", "set", "end"}."get", "queue_name"=w339) -> ("queue_out"=w343:refnum<queue>)  [unwired: 5 in, 4 out]
                n128 = To Variant() -> (Variant=w342:variant)  [unwired: 1 in]
                n129 = Unbundle By Name(w345) -> ()  [unwired: 1 out]
                n130 = Enqueue Element(queue=w343, element=w342, timeout in ms (-1)=100 ("超时毫秒(-1)")) -> ()  [unwired: 1 in, 3 out]
                n131 = property on="CFX_Message_In" class="Clust (严格)" props=["Value"]() -> ()  [unwired: 2 in, 3 out]
                n132 = property on="CFX_Message_In" class="Clust (严格)" props=["Value"](error in=w346) -> (error out=w347:errorcluster)  [unwired: 2 in, 1 out]
                n133 = call <vilib>:"Clear Errors.vi"("error in (no error)"=w347) -> ()  [unwired: 5 in, 2 out]
              }
              frame Enabled {
              }
            }
          }
        }
        n134 = Equal?(x=w306, y=w299) -> (x = y?=w301:bool)
        n135 = Select(t=w306, s=w301, f=w299) -> (s? t:f=w285:T7)
        n136 = local read "MessageCFX_out"() -> (w305:string)
        n137 = Select(t=CFX-cmd."Shutdown" ("CFX State"), s=w274, f=w285) -> (s? t:f=w284:T7)
      }
      frame "Shutdown" {
        n138 = Equal?(x=CfxTopic-cmd."EndpointShuttingDown" ("CFX cmd"), y=w351) -> (x = y?=w349:bool)
        n139 = case shown="True" w349 {
          tunnel: w360 -> [w364 w371]
          tunnel: [_ "关闭CFX通讯" ("格式字符串")] -> w359
          tunnel: [CFX-cmd."CFX" ("CFX State") w368] -> w358
          tunnel: w357 -> [w362 w391]
          tunnel: w356 -> [w363 w373]
          tunnel: [w364 w370] -> w355
          tunnel: [w363 w372] -> w354
          tunnel: [w362 w369] -> w353
          tunnel: [_ TRUE] -> w352
          tunnel: [CfxTopic-cmd."EndpointShuttingDown" ("CFX cmd") _] -> w348
          frame False {
          }
          frame True {
            n140 = invoke on="调用节点" class="AmqpCFXEndpoint" method="Close"(reference=w373, error in=w391) -> (reference out=w394:refnum<k24>, error out=w395:errorcluster)  [unwired: 1 in, 1 out]
            n141 = invoke on="调用节点" class="AmqpCFXEndpoint" method="Dispose"(reference=w394, error in=w395) -> (reference out=w372:refnum<k24>, error out=w390:errorcluster)  [unwired: 1 in, 1 out]
            n142 = invoke on="调用节点" class="AmqpCFXEndpoint" method="Close"(reference=w371, error in=w390) -> (reference out=w388:refnum<k24>, error out=w389:errorcluster)  [unwired: 1 in, 1 out]
            n143 = invoke on="调用节点" class="AmqpCFXEndpoint" method="Dispose"(reference=w388, error in=w389) -> (reference out=w370:refnum<k24>, error out=w387:errorcluster)  [unwired: 1 in, 1 out]
            n144 = Close Reference(reference=w372, error in (no error)=w387) -> (error out=w386:errorcluster)
            n145 = Close Reference(reference=w370, error in (no error)=w386) -> (error out=w381:errorcluster)
            n146 = call <vilib>:"Clear Errors.vi"("error in (no error)"=w381) -> ("error out"=w380:errorcluster)  [unwired: 5 in, 1 out]
            n147 = property on="TraceMessage_EVE" class="Ref (严格)"(error in=w380) -> (error out=w384:errorcluster, "Value"=w385:refnum<k27>)  [unwired: 1 in, 1 out]
            n148 = Unregister For Events(event registration refnum=w385, error in=w384) -> (error out=w379:errorcluster)
            n149 = property on="objAMQP_MSG" class="Ref (严格)"(error in=w379) -> (error out=w378:errorcluster, "Value"=w377:refnum<k27>)  [unwired: 1 in, 1 out]
            n150 = Unregister For Events(event registration refnum=w377, error in=w378) -> (error out=w376:errorcluster)
            n151 = property on="objAMQP_Request" class="Ref (严格)"(error in=w376) -> (error out=w375:errorcluster, "Value"=w374:refnum<k27>)  [unwired: 1 in, 1 out]
            n152 = property on="ok?" class="Bool (严格)"() -> ("Value"=w367:bool)  [unwired: 2 in, 2 out]
            n153 = Unregister For Events(event registration refnum=w374, error in=w375) -> (error out=w383:errorcluster)
            n154 = call <vilib>:"Clear Errors.vi"("error in (no error)"=w383) -> ("error out"=w369:errorcluster)  [unwired: 5 in, 1 out]
            n155 = Select(t=CFX-cmd."Shutdown" ("CFX State"), s=w367, f=CFX-cmd."Initialize") -> (s? t:f=w368:T7)
          }
        }
      }
      frame "WorkComplete" {
        w420 = 0 items=["Completed", "Failed", ""] ("Result")
        n156 = constructor class="WorkStarted"(error in=w398) -> (reference out=w421:refnum<k24>, error out=w418:errorcluster)  [unwired: 2 in, 1 out]
        n157 = property class="WorkStarted"(reference=w421, error in=w418) -> (error out=w417:errorcluster, "TransactionID"=w419:refnum<k24>)  [unwired: 1 out]
        n158 = constructor class="WorkCompleted"(error in=w417) -> (reference out=w416:refnum<k24>, error out=w415:errorcluster)  [unwired: 2 in, 1 out]
        n159 = property class="WorkCompleted"(reference=w416, error in=w415, "Result"=w420, "TransactionID"=w419) -> (reference out=w406:refnum<k24>, error out=w414:errorcluster)
        n160 = constructor class="CFXEnvelope"() -> (reference out=w423:refnum<k24>, error out=w422:errorcluster)  [unwired: 3 in, 1 out]
        n161 = property class="CFXEnvelope"(reference=w423, error in=w422, "MessageBody"=w406) -> (reference out=w409:refnum<k24>, error out=w410:errorcluster, "MessageName"=w404:string)
        n162 = invoke class="AmqpCFXEndpoint" method="Publish"(reference=w412, error in=w414, "env"=w409) -> (reference out=w411:refnum<k24>, error out=w413:errorcluster)  [unwired: 1 in, 2 out]
        n163 = invoke on="调用节点" class="CFXJsonSerializer" method="SerializeObjectWithTypes"("o"=w406, "formatted"=TRUE) -> (reference out=w405:refnum<k24>, error out=w407:errorcluster, "SerializeObjectWithTypes"=w403:string)  [unwired: 3 in, 2 out]
        n164 = Close Reference(reference=w405, error in (no error)=w407) -> (error out=w401:errorcluster)
        n165 = Merge Errors(w413, w410) -> (w408:errorcluster)
        n166 = Format Into String(format string="\n-------- Message Content --------\n%s" ("格式字符串"), initial string=w404, error in=w401, w403) -> (resulting string=w400:string)  [unwired: 1 out]
      }
      frame "StationStateChanged" {
        n167 = constructor class="StationStateChanged"(error in=w426) -> (reference out=w446:refnum<k24>, error out=w445:errorcluster)  [unwired: 2 in, 1 out]
        n168 = local read "rngNewState"() -> (w440:i32)
        n169 = property class="StationStateChanged"(reference=w446, error in=w445, "NewState"=w440) -> (reference out=w432:refnum<k24>, error out=w442:errorcluster)
        n170 = constructor class="CFXEnvelope"() -> (reference out=w443:refnum<k24>, error out=w444:errorcluster)  [unwired: 3 in, 1 out]
        n171 = property class="CFXEnvelope"(reference=w443, error in=w444, "MessageBody"=w432) -> (reference out=w435:refnum<k24>, error out=w437:errorcluster, "MessageName"=w430:string)
        n172 = invoke class="AmqpCFXEndpoint" method="Publish"(reference=w441, error in=w442, "env"=w435) -> (reference out=w439:refnum<k24>, error out=w438:errorcluster)  [unwired: 1 in, 2 out]
        n173 = invoke on="调用节点" class="CFXJsonSerializer" method="SerializeObjectWithTypes"("o"=w432, "formatted"=TRUE) -> (reference out=w434:refnum<k24>, error out=w433:errorcluster, "SerializeObjectWithTypes"=w428:string)  [unwired: 3 in, 2 out]
        n174 = Close Reference(reference=w434, error in (no error)=w433) -> (error out=w429:errorcluster)
        n175 = Merge Errors(w438, w437) -> (w436:errorcluster)
        n176 = Format Into String(format string="\n-------- Message Content --------%s" ("格式字符串"), initial string=w430, error in=w429, w428) -> ()  [unwired: 2 out]
      }
      frame "MaterialsApplied" {
        n177 = constructor class="MaterialsApplied"(error in=w449) -> (reference out=w472:refnum<k24>, error out=w474:errorcluster)  [unwired: 2 in, 1 out]
        n178 = constructor class="InstalledMaterial"() -> (reference out=w470:refnum<k24>, error out=w471:errorcluster)  [unwired: 3 in, 1 out]
        n179 = invoke class="Guid" method="NewGuid"(error in=w474) -> (error out=w475:errorcluster, "NewGuid"=w473:refnum<k24>)  [unwired: 2 in, 1 out]
        n180 = property class="MaterialsApplied"(reference=w472, error in=w475, "TransactionId"=w473) -> (reference out=w481:refnum<k24>, error out=w462:errorcluster, "AppliedMaterials"=w476:refnum<k24>)
        n181 = property class="InstalledMaterial"(reference=w470, error in=w471, "QuantityInstalled"=1.0, "QuantityNonInstalled"=2.0) -> (reference out=w477:refnum<k24>, error out=w459:errorcluster)
        n182 = Merge Errors(w462, w459) -> (w460:errorcluster)
        n183 = invoke class="List`1[[CFX.Structures.Installe" method="Add"(reference=w476, error in=w460, "item"=w477) -> (reference out=w478:refnum<k24>, error out=w461:errorcluster)  [unwired: 1 in, 2 out]
        n184 = property class="MaterialsApplied"(reference=w481, error in=w461, "AppliedMaterials"=w478) -> (reference out=w455:refnum<k24>, error out=w463:errorcluster)
        n185 = constructor class="CFXEnvelope"(error in=w463) -> (reference out=w479:refnum<k24>, error out=w480:errorcluster)  [unwired: 2 in, 1 out]
        n186 = property class="CFXEnvelope"(reference=w479, error in=w480, "MessageBody"=w455) -> (reference out=w458:refnum<k24>, error out=w464:errorcluster, "MessageName"=w453:string)
        n187 = invoke class="AmqpCFXEndpoint" method="Publish"(reference=w467, error in=w464, "env"=w458) -> (reference out=w466:refnum<k24>, error out=w465:errorcluster)  [unwired: 1 in, 2 out]
        n188 = invoke on="调用节点" class="CFXJsonSerializer" method="SerializeObjectWithTypes"("o"=w455, "formatted"=TRUE) -> (reference out=w456:refnum<k24>, error out=w457:errorcluster, "SerializeObjectWithTypes"=w452:string)  [unwired: 3 in, 2 out]
        n189 = Close Reference(reference=w456, error in (no error)=w457) -> ()  [unwired: 1 out]
        n190 = Format Into String(format string="\n-------- Message Content --------\n%s" ("格式字符串"), initial string=w453, w452) -> (resulting string=w451:string)  [unwired: 1 in, 1 out]
      }
      frame "CFX" {
        w486 = CfxTopic-cmd."EndpointShuttingDown" ("CFX cmd")
        n191 = First Call?() -> (First Call?: T/F=w496:bool)
        n192 = Not Equal?(x=w491, y=CfxTopic-cmd."AreYouThereRequest" ("CFX cmd")) -> (x != y?=w497:bool)
        n193 = property on="return" class="Clust (严格)"() -> ("Value"=w495:T5)  [unwired: 2 in, 2 out]
        n194 = Equal?(x=w486, y=w491) -> (x = y?=w490:bool)
        n195 = Or(x=w497, y=w496) -> (x .or. y?=w498:bool)
        n196 = Unbundle By Name(w495) -> ("CFXHandle"=w494:string, "RequestNetworkUri"=w493:string, "RequestTargetAddress"=w492:string)
        n197 = case shown="True" w498 {
          tunnel: w491 -> [_ w520]
          tunnel: ["CFX cmd" w520] -> w499
          frame False {
          }
          frame True {
          }
        }
        n198 = property on="EndpointInformation" class="Str"(error in=w509) -> (error out=w514:errorcluster, "Value"=w517:string)  [unwired: 1 in, 1 out]
        n199 = call "_lcod_CFX.vi"("RequestTargetAddress"=w492, "RequestNetworkUri"=w493, "cmd"=w499, "Error In"=w514, "in_str"=w517, "CFXHandle"=w494, "CfxData"="CfxData") -> ("Error Out"=w485:errorcluster, "new reference"=w504:refnum<k24>)  [unwired: 2 in, 1 out]
        n200 = Get Date/Time In Seconds() -> (seconds since 1Jan1904=w510:timestamp)
        n201 = property class="CFXEnvelope" props=["CFXVERSION", "MessageName", "Source", "Target", "TimeStamp"](reference=w504, error in=w485, "Source"=w484, "Target"=w483, "TimeStamp"=w510) -> (reference out=w503:refnum<k24>, error out=w511:errorcluster, "MessageName"=w502:string)  [unwired: 1 out]
        n202 = invoke class="AmqpCFXEndpoint" method="Publish"(reference=w508, error in=w511, "env"=w503) -> (reference out=w506:refnum<k24>, error out=w518:errorcluster)  [unwired: 1 in, 2 out]
        n203 = invoke on="调用节点" class="CFXJsonSerializer" method="SerializeObjectWithTypes"("o"=w503, "formatted"=TRUE) -> (reference out=w515:refnum<k24>, error out=w516:errorcluster, "SerializeObjectWithTypes"=w501:string)  [unwired: 3 in, 2 out]
        n204 = Close Reference(reference=w515, error in (no error)=w516) -> ()  [unwired: 1 out]
        n205 = Format Into String(format string="Direction: Send | %s\n-------- Message Content -------\n%s" ("格式字符串"), w502, w501) -> (resulting string=w512:string)  [unwired: 2 in, 1 out]
        n206 = Select(t=CFX-cmd."Shutdown" ("CFX State"), s=w490, f=CFX-cmd."Idle" ("CFX State")) -> (s? t:f=w487:T7)
      }
      frame "Hermes" {
        n207 = disable-structure shown="禁用" {
          disable-tunnel: w527 -> [w530 w532]
          disable-tunnel: [w529 w532] -> w526
          disable-tunnel: [w528 w531] -> w525
          disable-tunnel: [_ ""] -> w524
          disable-tunnel: w522 -> [_ w531]
          frame Disabled {
            n208 = invoke class="AmqpCFXEndpoint" method="Publish"(reference=w530) -> (reference out=w529:refnum<k24>, error out=w528:errorcluster)  [unwired: 3 in, 2 out]
          }
          frame Enabled {
          }
        }
      }
    }
    "MessageCFX_out" <- w64
    n209 = Call Chain() -> (call chain=w46:string[])
    n210 = Array Size(array=w46) -> (size(s)=w45:i32)
    n211 = Empty String/Path?(string/path=w61) -> (empty?=w60:bool)
    n212 = disable-structure shown="禁用" {
      disable-tunnel: w41 -> [w68 _]
      frame Disabled {
        n213 = local write "CFX State"(w68) -> ()
      }
      frame Enabled {
      }
    }
    n214 = Equal?(x=w41, y=w26) -> (x = y?=w38:bool)
    n215 = Greater?(x=w45, y=1) -> (0:w39:bool)
    n216 = case shown="False" w60 {
      tunnel: w65 -> [w87 w89]
      tunnel: [w86 w88] -> w58
      tunnel: w61 -> [w81 _]
      tunnel: w30 -> [w79 _]
      frame False {
        n217 = call "Cfx_log.vi"("login"=w81, "error in"=w87, "log_path"=w79) -> ("Log_out"=w80:string, "error out"=w86:errorcluster)  [unwired: 15 in]
        n218 = Format Into String(format string="CFX . 执行信息】\n消息：%s", w80) -> (resulting string=w84:string, error out=w85:errorcluster)  [unwired: 2 in]
        n219 = call "lcod run log.vi"("cmd"=_myType_runlog_cmd."push (1: logical)", "Error In"=w85, "str in"=w84) -> ()  [unwired: 6 in, 3 out]
        "log" <- w81
      }
      frame True {
        n220 = call <vilib>:"Simple Error Handler.vi"("error in (no error)"=w89) -> ("error out"=w88:errorcluster)  [unwired: 4 in, 4 out]
      }
    }
    "error out" <- w58
    n221 = And(x=w38, y=w39) -> (x .and. y?=w40:bool)
    n222 = case shown="False" w40 {
      tunnel: w43 -> [w74 w76]
      tunnel: [w74 w77] -> w42
      tunnel: [_ w75] -> w28
      frame False {
        n223 = Wait (ms)(milliseconds to wait=u32 10 ("等待时间（毫秒）")) -> ()  [unwired: 1 out]
      }
      frame True {
        n224 = call "lcod exit.vi"() -> ("bExit out"=w75:bool)  [unwired: 11 in]
        n225 = Select(t=w76, s=w75, f=TRUE) -> (s? t:f=w77:bool)
      }
    }
  }
  n226 = Bundle By Name(cluster=w2, "CFX_Handle"=w3) -> (→"CFX_Message_In":T3)
  n227 = disable-structure shown="已启用" {
    frame Disabled {
      n228 = constructor class="EndpointConnected"() -> (reference out=w544:refnum<k24>, error out=w545:errorcluster)  [unwired: 3 in, 1 out]
      n229 = invoke class="Dns" method="GetHostName"() -> ()  [unwired: 3 in, 3 out]
      n230 = invoke class="Dns" method="GetHostName"() -> (error out=w549:errorcluster, "GetHostName"=w546:string)  [unwired: 3 in, 1 out]
      n231 = Concatenate Strings("amqp://") -> ()  [unwired: 1 in, 1 out]
      n232 = invoke on="调用节点" class="EndpointConnected" method="GetHashCode"(reference=w544, error in=w545) -> ()  [unwired: 1 in, 3 out]
      n233 = invoke on="调用节点" class="CFXJsonSerializer" method="DeserializeObject"() -> ()  [unwired: 5 in, 5 out]
      n234 = constructor class="UriFormat"(error in=w549) -> (reference out=w551:refnum<k24>, error out=w550:errorcluster)  [unwired: 2 in, 1 out]
      n235 = Concatenate Strings("amqp://localhost:5672/#/" ("format"), w546) -> (w547:string)
      n236 = property class="EndpointConnected" props=["RequestNetworkUri"]() -> ()  [unwired: 3 in, 2 out]
      n237 = invoke class="UriFormat" method="ToString"(reference=w551, error in=w550, "format"=w547) -> ()  [unwired: 1 in, 4 out]
      n238 = constructor class="AppLogSettings"() -> ()  [unwired: 3 in, 3 out]
      n239 = property class="CFXJsonSerializer" props=["JsonSettings"]() -> ()  [unwired: 3 in, 2 out]
      n240 = invoke on="调用节点" class="CFXJsonSerializer" method="SerializeObjectWithTypes"() -> (reference out=w542:refnum<k24>, error out=w543:errorcluster)  [unwired: 5 in, 3 out]
      n241 = call "lcod log for app error.vi"() -> ()  [unwired: 10 in, 2 out]
      n242 = Format Into String() -> ()  [unwired: 4 in, 2 out]
      n243 = Close Reference(reference=w542, error in (no error)=w543) -> ()  [unwired: 1 out]
      n244 = Format Into String(format string="-------- Message Content --------\n%s" ("格式字符串")) -> ()  [unwired: 3 in, 2 out]
      n245 = disable-structure shown="已启用" {
        disable-tunnel: [w557 w559] -> _
        disable-tunnel: [w556 w558] -> _
        disable-tunnel: _ -> [w555 w559]
        disable-tunnel: _ -> [w554 w558]
        frame Disabled {
          n246 = invoke class="AmqpCFXEndpoint" method="AddSubscribeChannel"(reference=w555, error in=w554) -> (reference out=w553:refnum<k24>, error out=w552:errorcluster)  [unwired: 4 in, 4 out]
          n247 = invoke class="AmqpCFXEndpoint" method="AddMessageSource"(reference=w553, error in=w552) -> (reference out=w557:refnum<k24>, error out=w556:errorcluster)  [unwired: 2 in, 2 out]
        }
        frame Enabled {
        }
      }
      n248 = property on="CFX_Message_In" class="Clust (严格)"() -> ("Value"=w537:T10)  [unwired: 2 in, 2 out]
      n249 = feedback #2() -> (w539:T10)  [unwired: 1 in]
      n250 = Not Equal?(x=w537, y=w539) -> ()  [unwired: 1 out]
      n251 = feedback-in #2(w537) -> ()
      n252 = To Variant() -> (anything=w536:cluster{}, Variant=w535:variant)
      n253 = call "locd_queue[].vi"("cmd"=enum16{"init", "get", "set", "end"}."get") -> ("queue_out"=w538:refnum<queue>)  [unwired: 6 in, 4 out]
      n254 = Enqueue Element(queue=w538, element=w535) -> ()  [unwired: 2 in, 3 out]
    }
    frame Enabled {
      n255 = disable-structure shown="已启用" {
        frame Disabled {
          n256 = local write item#-1("" ("strCFXHandle")) -> ()
        }
        frame Enabled {
        }
      }
    }
  }
  n257 = Merge Errors("Error In", w4) -> (→"Error Out":errorcluster)
